vi "DAC Configure.vi"(8 "error in":errorcluster, 11 "DAC HeatFlow AOV in":refnum<class "DAC HeatFlow AOV.lvclass">) -> (0 "error out":errorcluster, 3 "DAC HeatFlow AOV out":refnum<class "DAC HeatFlow AOV.lvclass">)   [LabVIEW 2019, in "DAC.lvlib" / "DAC HeatFlow AOV.lvclass"]
uses:
  DAC HeatFlow AOV.lvclass
  C:/Users/wg/Documents/LV_Projects/test-stand/App/DAC/DAC.lvclass
  DAC.lvclass/DAC.ctl
  DAC HeatFlow AOV.lvclass/DAC HeatFlow AOV.ctl
  <vilib>/DAQmx/create/channels.llb/DAQmx Create Channel (AO-Voltage-Basic).vi
  DAC.lvclass
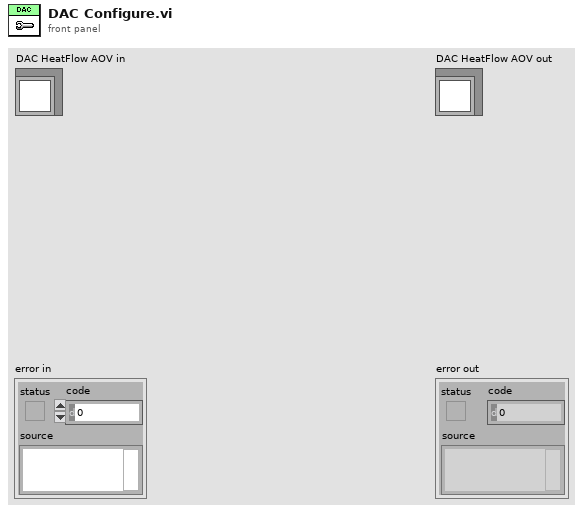
[diagram p1: front panel]
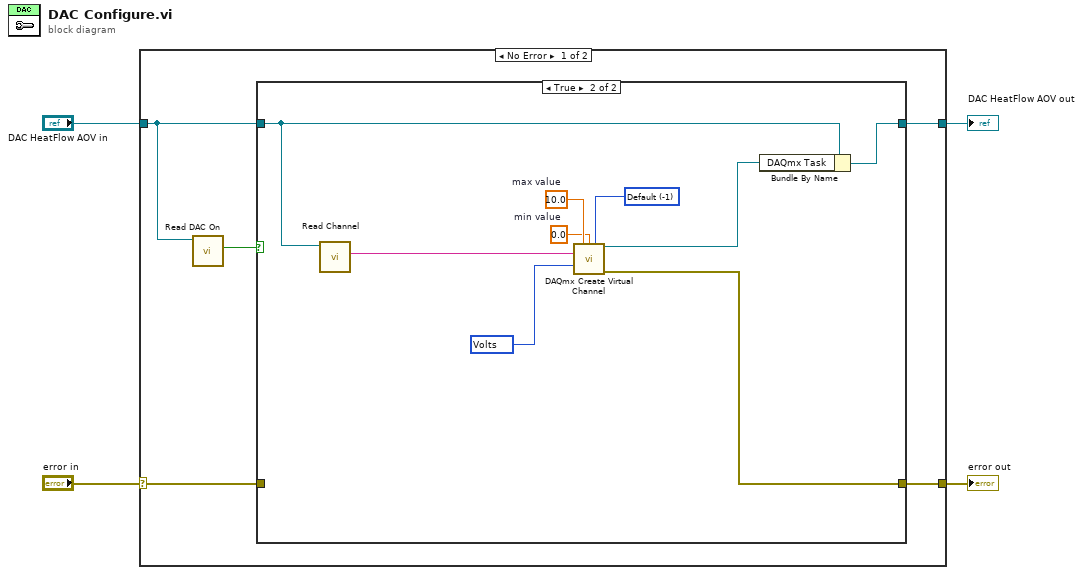
[diagram p0: block diagram]
diagram:
  n1 = case shown="No Error" "error in" {
    selector: "error in" -> [w6 w22]
    tunnel: [w5 w22] -> w4
    tunnel: [w7 w21] -> w3
    tunnel: "DAC HeatFlow AOV in" -> [w9 w21]
    frame No Error {
      n2 = call "Read DAC On.vi"("DAC in"=w9) -> ("DAC On"=w8:bool)  [unwired: 8 in, 2 out]
      n3 = case shown="True" w8 {
        tunnel: w9 -> [w11 w19]
        tunnel: [w11 w20] -> w7
        tunnel: w6 -> [w10 _]
        tunnel: [w10 w13] -> w5
        frame False {
        }
        frame True {
          w14 = 10348 items=["Volts"=10348, "From Custom Scale"=10065] ("units")
          w15 = -1 items=["Default"=-1, "RSE"=10083, "NRSE"=10078, "Differential"=10106, "Pseudodifferential"=12529] ("input terminal configuration")
          w16 = 0.0  # min value
          w17 = 10.0  # max value
          n4 = call "Read Channel.vi"("DAC in"=w19) -> ("Channel"=w12:string)  [unwired: 8 in, 2 out]
          n5 = call-poly <vilib>:"DAQmx Create Virtual Channel.vi"("maximum value"=w17, "minimum value"=w16, "output terminal configuration"=w15, "physical channels"=w12, "units"=w14) -> ("task out"=w18:refnum<k21>, "error out"=w13:errorcluster)  [unwired: 9 in]
          n6 = Bundle By Name(cluster=w19, "DAQmx Task"=w18) -> (w20:refnum<class "DAC HeatFlow AOV.lvclass">)
        }
      }
    }
    frame Error {
    }
  }
  "error out" <- w4
  "DAC HeatFlow AOV out" <- w3
